vi "CSE ISP - set VI title.vi"(7 "include full path?":bool, 8 "error in":errorcluster, 10 "script path":path, 11 "vi RefNum":refnum<vi>) -> (0 "error out":errorcluster, 3 "dup vi RefNum":refnum<vi>)   [LabVIEW 2021]
doc: "::: CalcExpress Toolkit :::\nCopyright (c) 2000-2026 Konstantin Shifershteyn. All rights reserved."
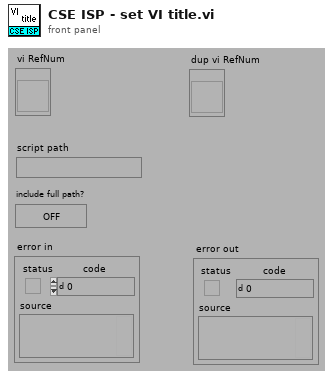
[diagram p1: front panel]
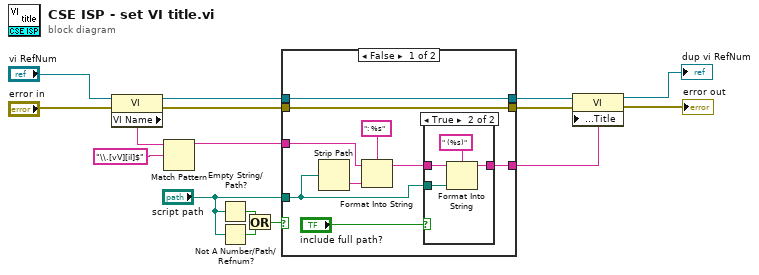
[diagram p0: block diagram]
diagram:
  n1 = property class="VI"(reference="vi RefNum", error in="error in") -> (reference out=w7:refnum<vi>, error out=w6:errorcluster, "VI Name"=w3:string)
  n2 = Match Pattern(string=w3, regular expression="\\.[vV][iI]$") -> (before substring=w1:string)  [unwired: 1 in, 3 out]
  n3 = Empty String/Path?(string/path="script path") -> (empty?=w11:bool)
  n4 = Not A Number/Path/Refnum?(number/path/refnum="script path") -> (NaN/Path/Refnum?=w10:bool)
  n5 = Or(x=w11, y=w10) -> (x .or. y?=w12:bool)
  n6 = case shown="False" w12 {
    tunnel: w6 -> [w23 w32]
    tunnel: w7 -> [w24 w33]
    tunnel: [w24 w33] -> w16
    tunnel: [w23 w32] -> w15
    tunnel: "script path" -> [w19 _]
    tunnel: [w20 w31] -> w8
    tunnel: w1 -> [w17 w31]
    frame False {
      n7 = Strip Path(path=w19) -> (name=w22:string)  [unwired: 1 out]
      n8 = Format Into String(format string=": %s", initial string=w17, w22) -> (resulting string=w21:string)  [unwired: 1 in, 1 out]
      n9 = case shown="True" "include full path?" {
        tunnel: [w26 w28] -> w20
        tunnel: w21 -> [w26 w29]
        tunnel: w19 -> [_ w27]
        frame False {
        }
        frame True {
          n10 = Format Into String(format string=" (%s)", initial string=w29, w27) -> (resulting string=w28:string)  [unwired: 1 in, 1 out]
        }
      }
    }
    frame True {
    }
  }
  n11 = property class="VI"(reference=w16, error in=w15, "Front Panel Window:Title"=w8) -> (reference out=→"dup vi RefNum":refnum<vi>, error out=→"error out":errorcluster)
